vi "RemoteVI Check Token Check.vi"() -> (4 "labels":string[](array[string]), 6 "expected":string[](array[string]), 8 "actual":string[](array[string]), 10 "failures":i32)   [LabVIEW 2020]
doc: "Test support, generated by tests/caraya/build.py from tests/vectors/http.json (tokens) - do not edit. Calls RemoteVI Token Check.vi once per vector: query and token as in the vector (the vector's token, or empty for emptyToken); ok? is rendered T or F. Outputs, one element per vector: labels (the vector's name), expected (rendered from the vector), actual (the VI's result rendered the same way), and failures, the number of vectors whose expected and actual differ."
uses:
  source/RemoteVI.lvlib
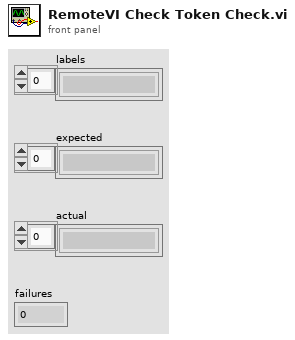
[diagram p1: front panel]
types:
  T1 = cluster{"name":string, "query":string, "token":string, "expect":string}[]
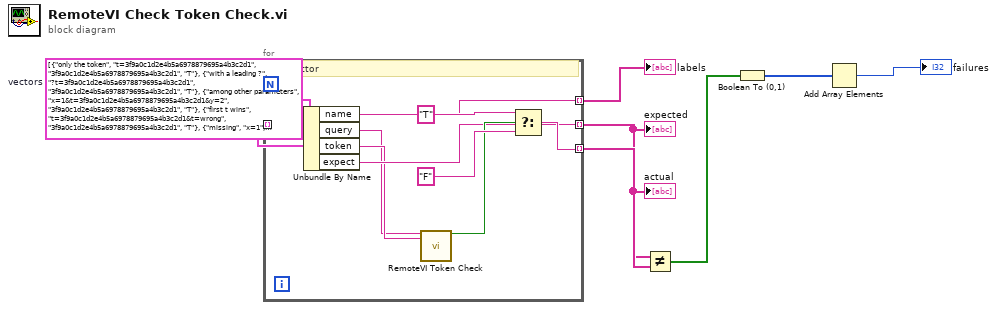
[diagram p0: block diagram]
diagram:
  w1 = T1 [{"name"="only the token", "query"="t=3f9a0c1d2e4b5a6978879695a4b3c2d1", "token"="3f9a0c1d2e4b5a6978879695a4b3c2d1", "expect"="T"}, {"name"="with a leading ?", "query"="?t=3f9a0c1d2e4b5a6978879695a4b3c2d1", "token"="3f9a0c1d2e4b5a6978879695a4b3c2d1", "expect"="T"}, {"name"="among other parameters", "query"="x=1&t=3f9a0c1d2e4b5a6978879695a4b3c2d1&y=2", "token"="3f9a0c1d2e4b5a6978879695a4b3c2d1", "expect"="T"}, {"name"="first t wins", "query"="t=3f9a0c1d2e4b5a6978879695a4b3c2d1&t=wrong", "token"="3f9a0c1d2e4b5a6978879695a4b3c2d1", "expect"="T"}, {"name"="missing", "query"="x=1", "token"="3f9a0c1d2e4b5a6978879695a4b3c2d1", "expect"="F"}, {"name"="empty query", "query"="", "token"="3f9a0c1d2e4b5a6978879695a4b3c2d1", "expect"="F"}, {"name"="wrong token", "query"="t=3f9a0c1d2e4b5a6978879695a4b3c2d2", "token"="3f9a0c1d2e4b5a6978879695a4b3c2d1", "expect"="F"}, {"name"="prefix only", "query"="t=3f9a0c1d", "token"="3f9a0c1d2e4b5a6978879695a4b3c2d1", "expect"="F"}, {"name"="longer", "query"="t=3f9a0c1d2e4b5a6978879695a4b3c2d100", "token"="3f9a0c1d2e4b5a6978879695a4b3c2d1", "expect"="F"}, {"name"="empty value", "query"="t=", "token"="3f9a0c1d2e4b5a6978879695a4b3c2d1", "expect"="F"}, {"name"="other key ending in t", "query"="at=3f9a0c1d2e4b5a6978879695a4b3c2d1", "token"="3f9a0c1d2e4b5a6978879695a4b3c2d1", "expect"="F"}, {"name"="uppercase key", "query"="T=3f9a0c1d2e4b5a6978879695a4b3c2d1", "token"="3f9a0c1d2e4b5a6978879695a4b3c2d1", "expect"="F"}, {"name"="empty token never matches", "query"="t=", "token"="", "expect"="F"}]  # vectors
  n1 = for {
    tunnel: w1 -> [w8] mode=indexing
    tunnel: [w9] -> w2 mode=indexing
    tunnel: [w12] -> w3 mode=indexing
    tunnel: [w16] -> w4 mode=indexing
    # "One vector"
    n2 = Unbundle By Name(w8) -> ("name"=w9:string, "query"=w10:string, "token"=w11:string, "expect"=w12:string)
    n3 = call "RemoteVI Token Check.vi"("query"=w10, "token"=w11) -> ("ok?"=w13:bool)  [unwired: 13 in]
    n4 = Select(t="T", s=w13, f="F") -> (s? t:f=w16:string)
  }
  "labels" <- w2
  "expected" <- w3
  "actual" <- w4
  n5 = Not Equal?(x=w3, y=w4) -> (x != y?=w5:bool[])
  n6 = Boolean To (0,1)(Boolean=w5) -> (0, 1=w6:i16[])
  n7 = Add Array Elements(numeric array=w6) -> (sum=→"failures":i16)
